vi "RemoteVI Wait Popup Age.vi"(0 "popup since":u32, 11 "error in":errorcluster) -> (15 "error out":errorcluster)   [LabVIEW 2020, in "RemoteVI.lvlib"]
doc: "Waits until the open popup is 350 ms old (popup since = tick count when the server first saw it) before a mouse-path click is posted to it: LabVIEW ignored clicks on a freshly opened ring menu (measured with posted messages: 200 ms ignored, 250 ms taken). Returns at once when the popup is older. Menus are clicked with keys, which LabVIEW takes right after a menu opened (measured: VK_DOWN 70 ms after the plot legend menu appeared), so only the mouse path waits. An incoming error is passed through; it does not skip the wait."
uses:
  RemoteVI.lvlib
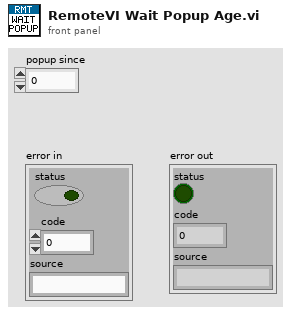
[diagram p1: front panel]
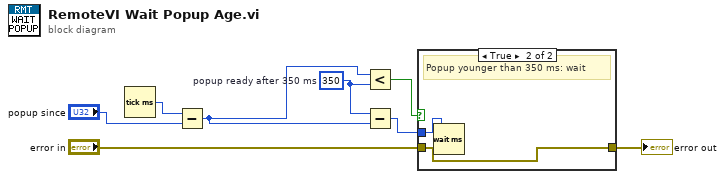
[diagram p0: block diagram]
diagram:
  w5 = u32 350  # popup ready after 350 ms
  n1 = Tick Count (ms)() -> (millisecond timer value=w3:u32)
  n2 = Subtract(x=w3, y="popup since") -> (x-y=w4:u32)
  n3 = Less?(x=w4, y=w5) -> (x < y?=w6:bool)
  n4 = Subtract(x=w5, y=w4) -> (x-y=w7:u32)
  n5 = case shown="True" w6 {
    tunnel: "error in" -> [w9 w10]
    tunnel: [w9 w10] -> w8
    tunnel: w7 -> [_ w11]
    frame False {
    }
    frame True {
      # "Popup younger than 350 ms: wait"
      n6 = Wait (ms)(milliseconds to wait=w11) -> ()  [unwired: 1 out]
    }
  }
  "error out" <- w8
